vi "hello.vi"(11 "input string":string="hello world" caption="experiment status text") -> (3 "resulting string":string="hello world" caption="validated status text")   [LabVIEW 2021]
doc: "Deterministic self-test VI for scientific automation via MCP. Use it before acquisition, analysis, or instrument-control workflows. Input a short experiment status string. The output returns exactly the same text unchanged so the LLM can verify LabVIEW-MCP connectivity and reproducible string IO without side effects."
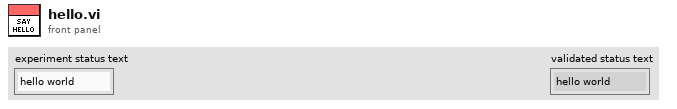
[diagram p1: front panel]
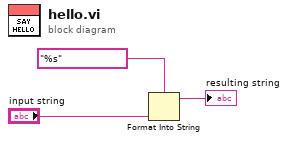
[diagram p0: block diagram]
diagram:
  n1 = Format Into String(format string="%s", "input string") -> (resulting string=→"resulting string":string)  [unwired: 2 in, 1 out]
